vi "Table_AssertColumnValue_Tests.vi"(8 "error in":errorcluster) -> (0 "error out":errorcluster)   [LabVIEW 2016, in "DronaTest.lvlib"]
uses:
  DronaTest.lvlib
  APIs/Stimulus/ControlValue/SetValueAuto.vi
  APIs/Assert/AssertControlValue/Controls/Table/AssertColumnValue.vi
  <vilib>/addons/_JKI Toolkits/Caraya/classes/Assert/Assert Equal Value_Variant.vi
  <vilib>/addons/_JKI Toolkits/Caraya/classes/Test/Test.lvclass
  <vilib>/SLL Toolkit/SLL Debug/SLL Debug.lvlib
  Drona.lvlib
  <vilib>/addons/_JKI Toolkits/Caraya/classes/Assert/Assert.lvclass
  APIs/Get/GetControlRef/GetControlRef.lvlib
  APIs/Assert/AssertControlValue/Controls/Table/AssertTable.lvlib
  APIs/Stimulus/ControlValue/ControlValue.lvlib
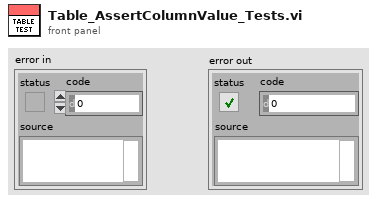
[diagram p1: front panel]
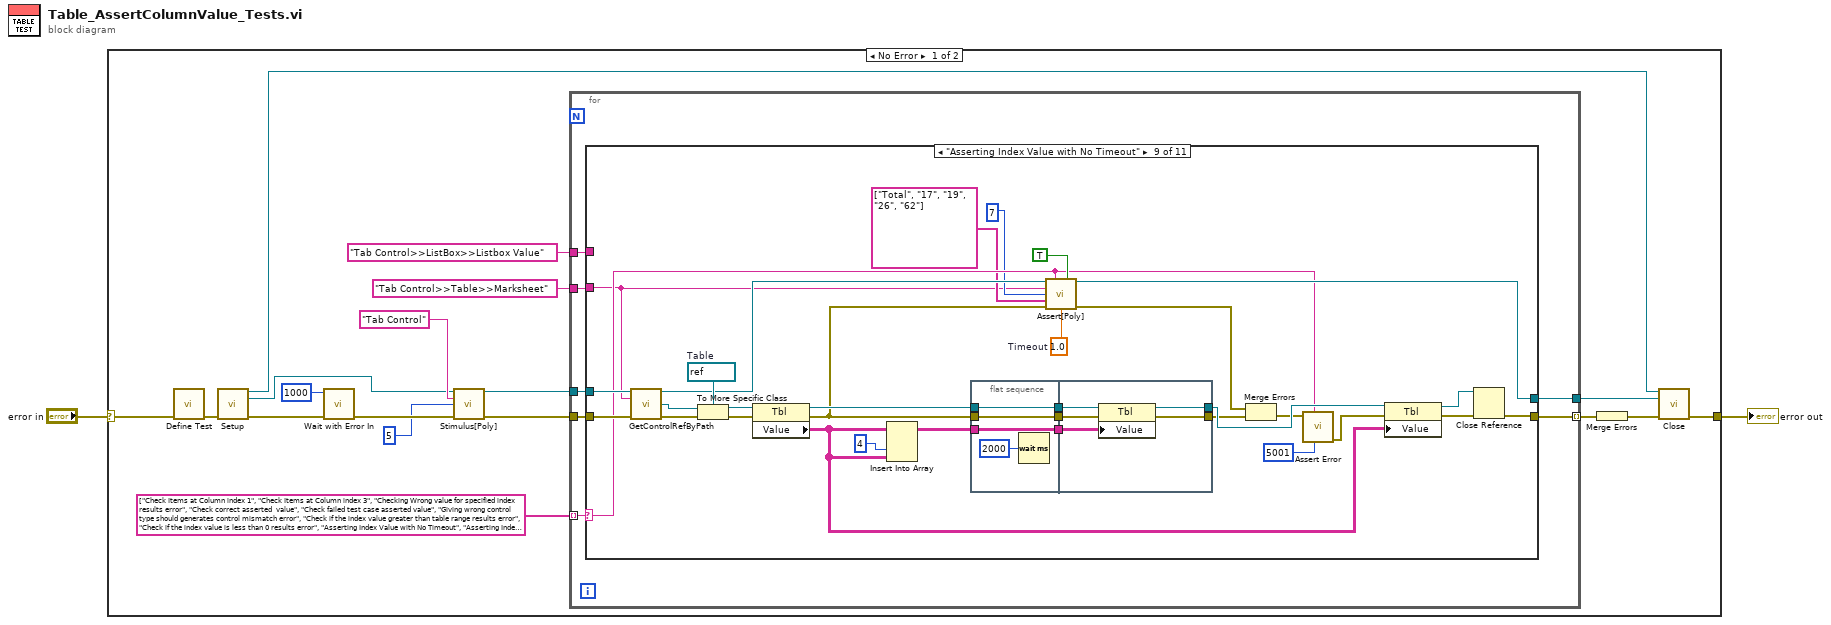
[diagram p0: block diagram]
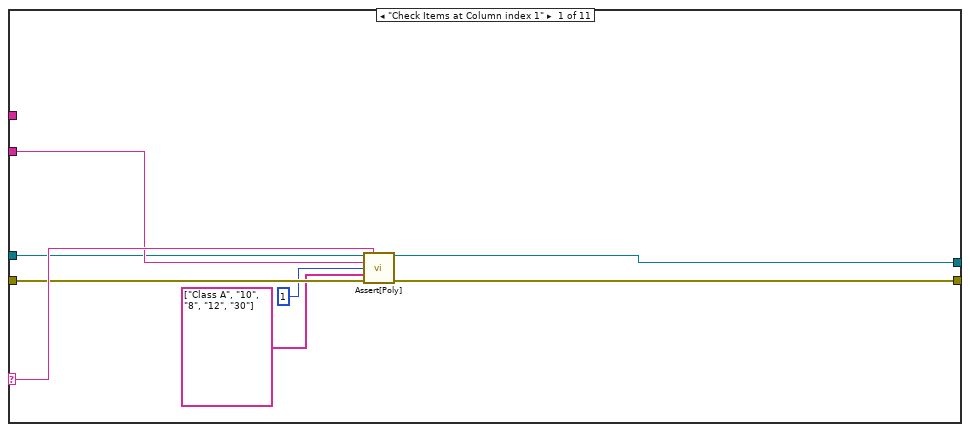
[diagram p2: hidden frame]
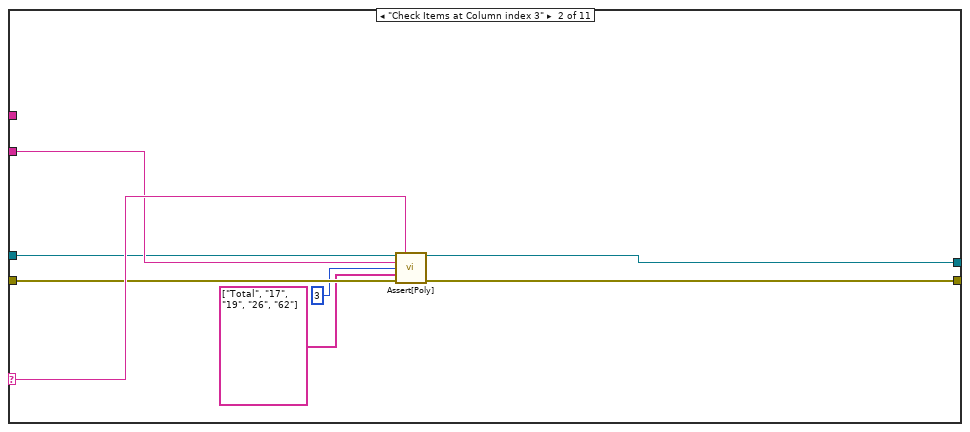
[diagram p3: hidden frame]
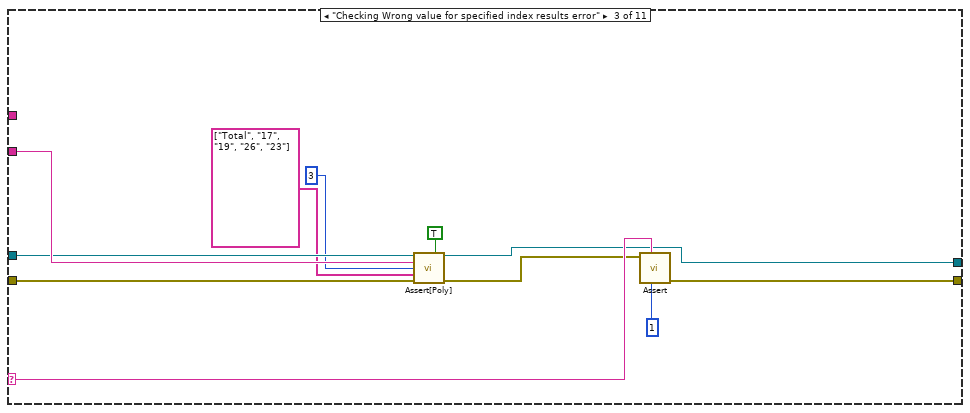
[diagram p4: hidden frame]
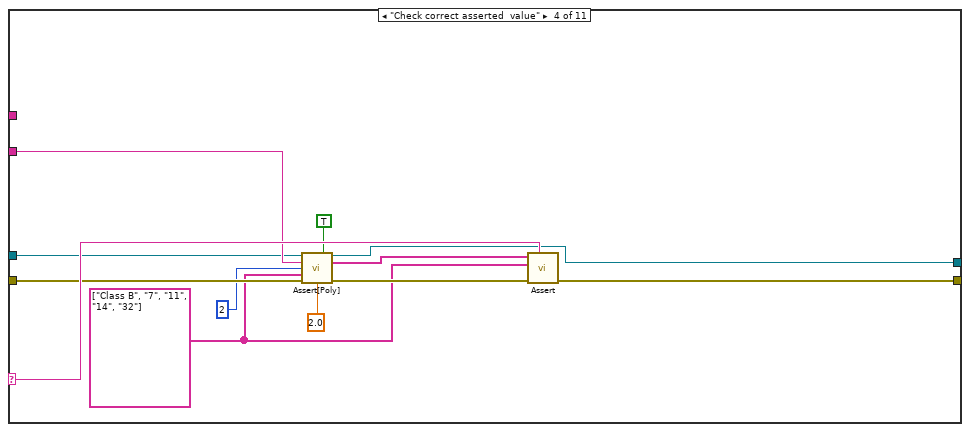
[diagram p5: hidden frame]
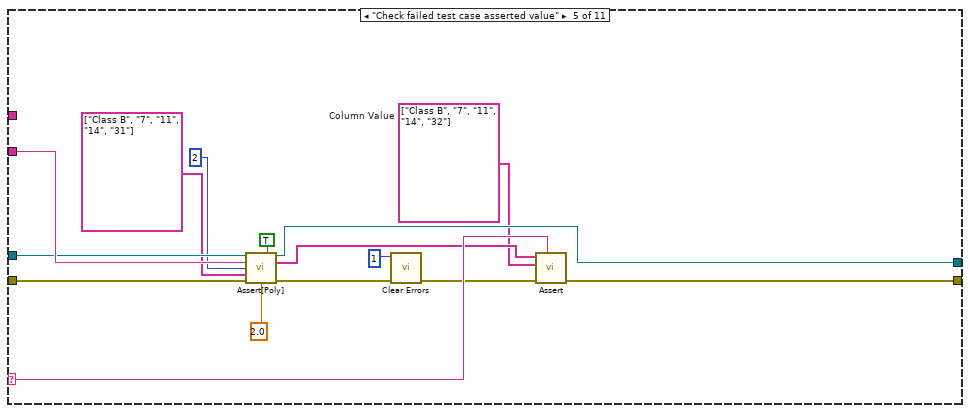
[diagram p6: hidden frame]
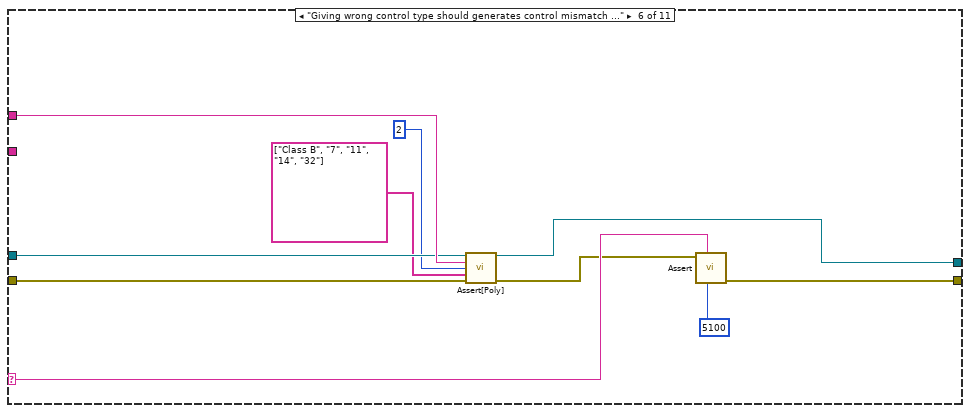
[diagram p7: hidden frame]
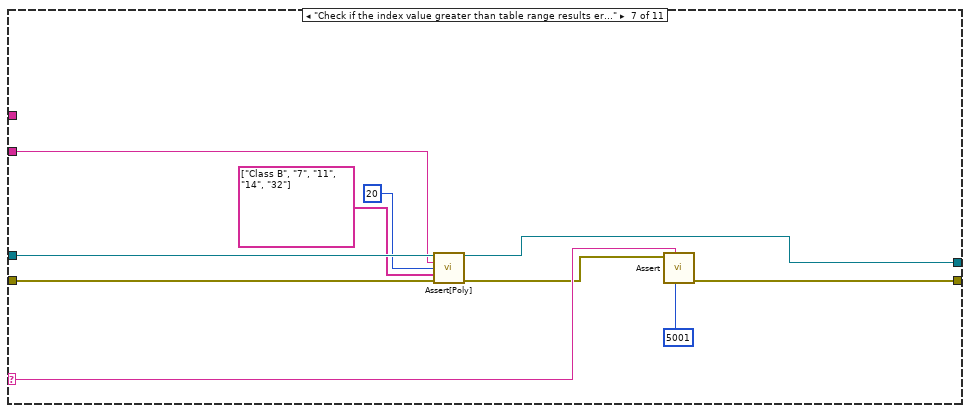
[diagram p8: hidden frame]
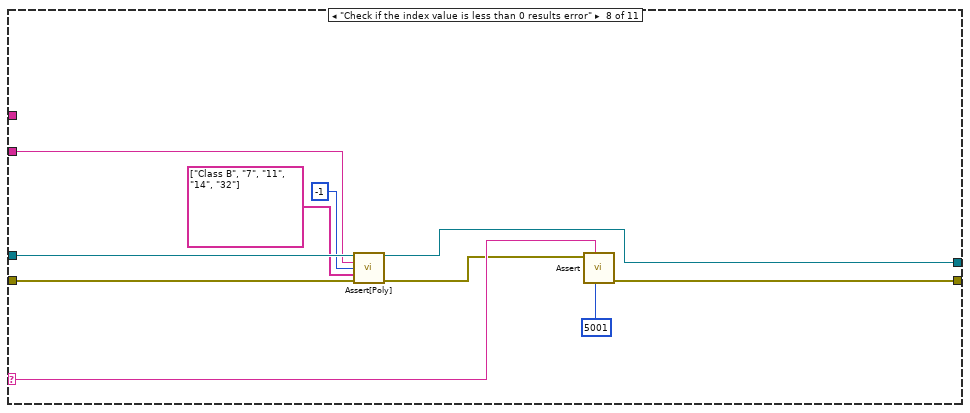
[diagram p9: hidden frame]
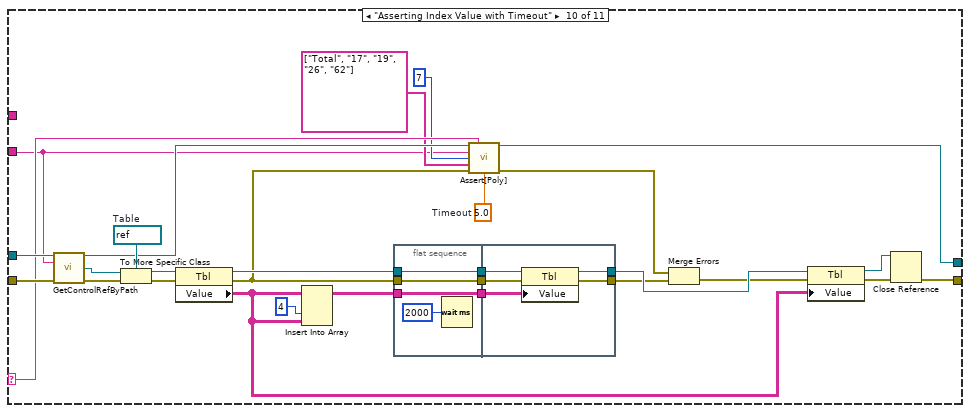
[diagram p10: hidden frame]
diagram:
  n1 = case shown="No Error" "error in" {
    selector: "error in" -> [w20 w193]
    tunnel: [w3 w193] -> w1
    frame No Error {
      n2 = call <vilib>:"Define Test.vi"("error in (no error)"=w20) -> ("error out"=w9:errorcluster)  [unwired: 9 in, 1 out]
      n3 = call "Setup.vi"("error in"=w9) -> ("Application Ref"=w5:refnum<vi>, "VI Reference Out"=w7:refnum<vi>, "error out"=w8:errorcluster)  [unwired: 12 in]
      n4 = call <vilib>:"Wait with Error In.vi"("error in (no error)"=w8, "milliseconds to wait"=u32 1000) -> ("error out"=w18:errorcluster)  [unwired: 9 in]
      n5 = call-poly "Stimulus[Poly].vi"("VI Reference In"=w7, "Control Path"="Tab Control", "Value (Signaling)"=5, "error in"=w18) -> ("VI Reference Out"=w14:refnum<vi>, "error out"=w17:errorcluster)  [unwired: 10 in]
      n6 = for {
        tunnel: w14 -> [w23]
        tunnel: "Tab Control>>Table>>Marksheet" ("Control Path") -> [w21]
        tunnel: "Tab Control>>ListBox>>Listbox Value" ("Control Path") -> [w22]
        tunnel: string[] ["Check Items at Column index 1", "Check Items at Column index 3", "Checking Wrong value for specified index results error", "Check correct asserted  value", "Check failed test case asserted value", "Giving wrong control type should generates control mismatch error", "Check if the index value greater than table range results error", "Check if the index value is less than 0 results error", "Asserting Index Value with No Timeout", "Asserting Index Value with Timeout"] -> [w27] mode=indexing
        tunnel: [w25] -> w4
        tunnel: w17 -> [w24]
        tunnel: [w26] -> w10 mode=indexing
        n7 = case shown="\"Asserting Index Value with No Timeout\"" w27 {
          selector: w27 -> [w33 w41 w53 w65 w80 w90 w100 w110 w118 w171 _]
          tunnel: w24 -> [w31 w39 w47 w61 w76 w85 w96 w106 w143 w181 w192]
          tunnel: w23 -> [w30 w38 w46 w60 w75 w84 w95 w105 w141 w179 w191]
          tunnel: w21 -> [w32 w40 w51 w64 w79 _ w94 w104 w112 w153 _]
          tunnel: w22 -> [_ _ _ _ _ w87 _ _ _ _ _]
          tunnel: [w35 w43 w54 w66 w81 w91 w101 w111 w130 w167 w192] -> w26
          tunnel: [w34 w42 w50 w63 w78 w86 w97 w107 w134 w172 w191] -> w25
          frame "Check Items at Column index 1" {
            n8 = call-poly "Assert[Poly].vi"("VI Reference In"=w30, "Test Label"=w33, "Control Path"=w32, "Column Index"=1 ("Item Index"), "Item Value"=string[] ["Class A", "10", "8", "12", "30"] ("Column Value"), "Error In"=w31) -> ("VI Reference Out"=w34:refnum<vi>, "Error Out"=w35:errorcluster)  [unwired: 7 in, 1 out]
          }
          frame "Check Items at Column index 3" {
            n9 = call-poly "Assert[Poly].vi"("VI Reference In"=w38, "Test Label"=w41, "Control Path"=w40, "Column Index"=3 ("Item Index"), "Item Value"=string[] ["Total", "17", "19", "26", "62"] ("Column Value"), "Error In"=w39) -> ("VI Reference Out"=w42:refnum<vi>, "Error Out"=w43:errorcluster)  [unwired: 7 in, 1 out]
          }
          frame "Checking Wrong value for specified index results error" {
            n10 = call-poly "Assert[Poly].vi"("VI Reference In"=w46, "Assert Only? (F)"=TRUE, "Control Path"=w51, "Column Index"=3 ("Item Index"), "Item Value"=string[] ["Total", "17", "19", "26", "23"] ("Column Value"), "Error In"=w47) -> ("VI Reference Out"=w50:refnum<vi>, "Error Out"=w49:errorcluster)  [unwired: 7 in, 1 out]
            n11 = call-poly <vilib>:"Assert.vi"("error code (1)"=1, "Label"=w53, "Error?"=w49) -> ("error out"=w54:errorcluster)  [unwired: 7 in, 1 out]
          }
          frame "Check correct asserted  value" {
            w55 = string[] ["Class B", "7", "11", "14", "32"] ("Column Value")
            n12 = call-poly "Assert[Poly].vi"("VI Reference In"=w60, "Assert Only? (F)"=TRUE, "Control Path"=w64, "Column Index"=2 ("Item Index"), "Item Value"=w55, "Error In"=w61, "Timeout(5 sec)"=2.0) -> ("VI Reference Out"=w63:refnum<vi>, "Asserted Value"=w58:string[], "Error Out"=w59:errorcluster)  [unwired: 6 in]
            n13 = call-poly <vilib>:"Assert.vi"("Label"=w65, "error in (no error)"=w59, "Y"=w55, "X"=w58) -> ("error out"=w66:errorcluster)  [unwired: 6 in, 1 out]
          }
          frame "Check failed test case asserted value" {
            w67 = string[] ["Class B", "7", "11", "14", "32"]  # Column Value
            n14 = call-poly "Assert[Poly].vi"("VI Reference In"=w75, "Assert Only? (F)"=TRUE, "Control Path"=w79, "Column Index"=2 ("Item Index"), "Item Value"=string[] ["Class B", "7", "11", "14", "31"] ("Column Value"), "Error In"=w76, "Timeout(5 sec)"=2.0) -> ("VI Reference Out"=w78:refnum<vi>, "Asserted Value"=w73:string[], "Error Out"=w74:errorcluster)  [unwired: 6 in]
            n15 = call <vilib>:"Clear Errors.vi"("error in (no error)"=w74, "specific error code to clear (0: all)"=1) -> ("error out"=w72:errorcluster)  [unwired: 4 in, 1 out]
            n16 = call-poly <vilib>:"Assert.vi"("Label"=w80, "error in (no error)"=w72, "Y"=w67, "X"=w73) -> ("error out"=w81:errorcluster)  [unwired: 6 in, 1 out]
          }
          frame "Giving wrong control type should generates control mismatch error" {
            n17 = call-poly "Assert[Poly].vi"("VI Reference In"=w84, "Control Path"=w87, "Column Index"=2 ("Item Index"), "Item Value"=string[] ["Class B", "7", "11", "14", "32"] ("Column Value"), "Error In"=w85) -> ("VI Reference Out"=w86:refnum<vi>, "Error Out"=w88:errorcluster)  [unwired: 8 in, 1 out]
            n18 = call-poly <vilib>:"Assert.vi"("error code (1)"=5100, "Label"=w90, "Error?"=w88) -> ("error out"=w91:errorcluster)  [unwired: 7 in, 1 out]
          }
          frame "Check if the index value greater than table range results error" {
            n19 = call-poly "Assert[Poly].vi"("VI Reference In"=w95, "Control Path"=w94, "Column Index"=20 ("Item Index"), "Item Value"=string[] ["Class B", "7", "11", "14", "32"] ("Column Value"), "Error In"=w96) -> ("VI Reference Out"=w97:refnum<vi>, "Error Out"=w98:errorcluster)  [unwired: 8 in, 1 out]
            n20 = call-poly <vilib>:"Assert.vi"("error code (1)"=5001, "Label"=w100, "Error?"=w98) -> ("error out"=w101:errorcluster)  [unwired: 7 in, 1 out]
          }
          frame "Check if the index value is less than 0 results error" {
            n21 = call-poly "Assert[Poly].vi"("VI Reference In"=w105, "Control Path"=w104, "Column Index"=-1 ("Item Index"), "Item Value"=string[] ["Class B", "7", "11", "14", "32"] ("Column Value"), "Error In"=w106) -> ("VI Reference Out"=w107:refnum<vi>, "Error Out"=w108:errorcluster)  [unwired: 8 in, 1 out]
            n22 = call-poly <vilib>:"Assert.vi"("error code (1)"=5001, "Label"=w110, "Error?"=w108) -> ("error out"=w111:errorcluster)  [unwired: 7 in, 1 out]
          }
          frame "Asserting Index Value with No Timeout" {
            w127 = 1.0  # Timeout
            w138 = refnum<vi> refnum  # Table
            n23 = call "GetControlRefByPath.vi"("VI Reference In"=w141, "Control Path"=w112, "error In"=w143) -> ("VI Reference Out"=w135:refnum<vi>, "Ctl Refnum"=w139:refnum<vi>, "error out"=w142:errorcluster)  [unwired: 10 in]
            n24 = To More Specific Class(target class=w138, reference=w139, error in=w142) -> (specific class reference=w137:refnum<vi>, error out=w140:errorcluster)
            n25 = property class="Tbl"(reference=w137, error in=w140) -> (reference out=w133:refnum<vi>, error out=w126:errorcluster, "Value"=w114:string[][])
            n26 = Insert Into Array(array=w114, index (col)=4 ("disabled index (col)"), new element=w114) -> (w136:string[][])  [unwired: 1 in]
            n27 = flat-sequence {
              tunnel: w126 -> [w145]
              tunnel: w133 -> [w146]
              tunnel: w136 -> [w147]
              tunnel: [w147] -> w124
              tunnel: [w146] -> w123
              tunnel: [w145] -> w122
              tunnel: [w150] -> w129
              tunnel: [w148] -> w125
              tunnel: w124 -> [w152]
              tunnel: w123 -> [w151]
              tunnel: w122 -> [w149]
              frame #0 {
                n28 = Wait (ms)(milliseconds to wait=u32 2000) -> ()  [unwired: 1 out]
              }
              frame #1 {
                n29 = property class="Tbl"(reference=w151, error in=w149, "Value"=w152) -> (reference out=w150:refnum<vi>, error out=w148:errorcluster)
              }
            }
            n30 = call-poly "Assert[Poly].vi"("VI Reference In"=w135, "Test Label"=w118, "Assert Only? (F)"=TRUE, "Control Path"=w112, "Column Index"=7 ("Row Index"), "Item Value"=string[] ["Total", "17", "19", "26", "62"] ("Column Value"), "Error In"=w126, "Timeout(5 sec)"=w127) -> ("VI Reference Out"=w134:refnum<vi>, "Error Out"=w132:errorcluster)  [unwired: 5 in, 1 out]
            n31 = Merge Errors(w132, w125) -> (w121:errorcluster)
            n32 = call <vilib>:"Assert Error.vi"("error code (1)"=5001, "Label"=w118, "Error?"=w121) -> ("error out"=w120:errorcluster)  [unwired: 7 in, 1 out]
            n33 = property class="Tbl"(reference=w129, error in=w120, "Value"=w114) -> (reference out=w128:refnum<vi>, error out=w131:errorcluster)
            n34 = Close Reference(reference=w128, error in (no error)=w131) -> (error out=w130:errorcluster)
          }
          frame "Asserting Index Value with Timeout" {
            w158 = 5.0  # Timeout
            w176 = refnum<vi> refnum  # Table
            n35 = call "GetControlRefByPath.vi"("VI Reference In"=w179, "Control Path"=w153, "error In"=w181) -> ("VI Reference Out"=w173:refnum<vi>, "Ctl Refnum"=w177:refnum<vi>, "error out"=w180:errorcluster)  [unwired: 10 in]
            n36 = To More Specific Class(target class=w176, reference=w177, error in=w180) -> (specific class reference=w175:refnum<vi>, error out=w178:errorcluster)
            n37 = property class="Tbl"(reference=w175, error in=w178) -> (reference out=w170:refnum<vi>, error out=w164:errorcluster, "Value"=w157:string[][])
            n38 = Insert Into Array(array=w157, index (col)=4 ("disabled index (col)"), new element=w157) -> (w174:string[][])  [unwired: 1 in]
            n39 = flat-sequence {
              tunnel: w164 -> [w183]
              tunnel: w170 -> [w184]
              tunnel: w174 -> [w185]
              tunnel: [w185] -> w161
              tunnel: [w184] -> w160
              tunnel: [w183] -> w159
              tunnel: [w188] -> w166
              tunnel: [w186] -> w162
              tunnel: w161 -> [w190]
              tunnel: w160 -> [w189]
              tunnel: w159 -> [w187]
              frame #0 {
                n40 = Wait (ms)(milliseconds to wait=u32 2000) -> ()  [unwired: 1 out]
              }
              frame #1 {
                n41 = property class="Tbl"(reference=w189, error in=w187, "Value"=w190) -> (reference out=w188:refnum<vi>, error out=w186:errorcluster)
              }
            }
            n42 = call-poly "Assert[Poly].vi"("VI Reference In"=w173, "Test Label"=w171, "Control Path"=w153, "Column Index"=7 ("Row Index"), "Item Value"=string[] ["Total", "17", "19", "26", "62"] ("Column Value"), "Error In"=w164, "Timeout(5 sec)"=w158) -> ("VI Reference Out"=w172:refnum<vi>, "Error Out"=w169:errorcluster)  [unwired: 6 in, 1 out]
            n43 = Merge Errors(w169, w162) -> (w163:errorcluster)
            n44 = property class="Tbl"(reference=w166, error in=w163, "Value"=w157) -> (reference out=w165:refnum<vi>, error out=w168:errorcluster)
            n45 = Close Reference(reference=w165, error in (no error)=w168) -> (error out=w167:errorcluster)
          }
          frame Default {
          }
        }
      }
      n46 = Merge Errors(w10) -> (w6:errorcluster)
      n47 = call "Close.vi"("Application Ref"=w5, "VI Reference"=w4, "error in"=w6) -> ("error out"=w3:errorcluster)  [unwired: 12 in]
    }
    frame Error {
    }
  }
  "error out" <- w1
